vi "First.vi"(7 "Address":string, 8 "Error In":errorcluster) -> (0 "Error Out":errorcluster)   [LabVIEW 2018, in "Tests.lvlib" / "Known Hosts.lvlib"]
uses:
  Known Hosts.lvlib
  src/Toolkit/Known Hosts/Type Definitions/Get Results.ctl
  <vilib>/Utility/error.llb/Clear Errors.vi
  src/Toolkit/Known Hosts/Support/Create from Session.vi
  <vilib>/Utility/sysdir.llb/Get System Directory.vi
  src/Toolkit/Known Host/Support/Create from Known Hosts.vi
  src/Toolkit/Known Host/Support/Destroy to Known Hosts.vi
  src/Toolkit/Known Hosts/Support/Destroy to Session.vi
  <vilib>/addons/_JKI Toolkits/Caraya/classes/Test/Test.lvclass
  <vilib>/addons/_JKI Toolkits/Caraya/classes/Assert/Assert.lvclass
  src/Toolkit/Known Hosts/Known Hosts.lvclass
  Tests.lvlib
  src/Toolkit/Session/Session.lvclass
  src/Toolkit/Known Host/Known Host.lvclass
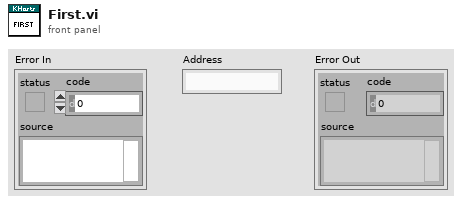
[diagram p1: front panel]
types:
  T1 = typedef "Toolkit.lvlib/Known Hosts.lvclass/Get Results.ctl" = i32
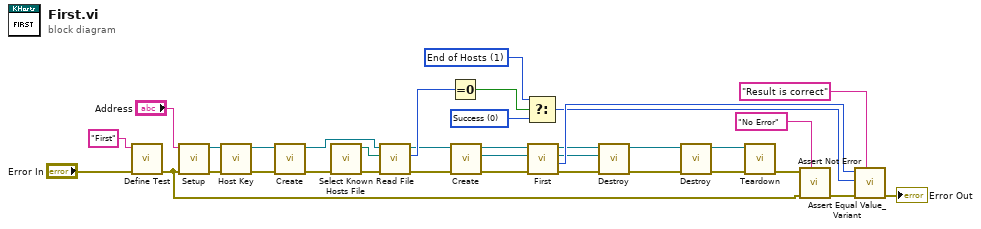
[diagram p0: block diagram]
diagram:
  w16 = T1 1 items=["Success", "End of Hosts"] ("Get Result")
  w17 = T1 0 items=["Success", "End of Hosts"] ("Get Result")
  n1 = call <vilib>:"Define Test.vi"("error in (no error)"="Error In", "Label (VI Title)"="First") -> ("error out"=w25:errorcluster)  [unwired: 9 in]
  n2 = call "Setup.vi"("Error In"=w25, "Address In"="Address") -> ("Error Out"=w26:errorcluster, "Sesssion"=w27:refnum<class "Session.lvclass">)  [unwired: 7 in, 1 out]
  n3 = call "Host Key.vi"("Error In"=w26, "Session In"=w27) -> ("Error Out"=w3:errorcluster, "Sesssion Out"=w4:refnum<class "Session.lvclass">)  [unwired: 6 in, 2 out]
  n4 = call-poly "Create.vi"("Error In"=w3, "Session"=w4) -> ("Error Out"=w2:errorcluster, "Known Hosts"=w1:refnum<class "Known Hosts.lvclass">)  [unwired: 8 in]
  n5 = call "Select Known Hosts File.vi"("Error In"=w2) -> ("Error Out"=w32:errorcluster, "Known Hosts File"=w31:path)  [unwired: 9 in]
  n6 = call "Read File.vi"("Error In"=w32, "File"=w31, "Known Hosts In"=w1) -> ("Error Out"=w22:errorcluster, "Count"=w19:u64, "Known Hosts Out"=w14:refnum<class "Known Hosts.lvclass">)  [unwired: 6 in]
  n7 = Equal To 0?(x=w19) -> (x = 0?=w18:bool)
  n8 = call-poly "Create.vi"("Error In"=w22, "Known Hosts In"=w14) -> ("Error Out"=w21:errorcluster, "Known Host"=w12:refnum<class "Known Host.lvclass">, "Known Hosts Out"=w13:refnum<class "Known Hosts.lvclass">)  [unwired: 7 in]
  n9 = Select(t=w16, s=w18, f=w17) -> (s? t:f=w15:T1)
  n10 = call "First.vi"("Error In"=w21, "Known Host In"=w12, "Known Hosts In"=w13) -> ("Error Out"=w9:errorcluster, "Result"=w20:T1, "Known Host Out"=w10:refnum<class "Known Host.lvclass">, "Known Hosts Out"=w11:refnum<class "Known Hosts.lvclass">)  [unwired: 5 in]
  n11 = call-poly "Destroy.vi"("Error In"=w9, "Known Host"=w10, "KnownHosts In"=w11) -> ("Error Out"=w5:errorcluster, "KnownHosts Out"=w8:refnum<class "Known Hosts.lvclass">)  [unwired: 7 in]
  n12 = call-poly "Destroy.vi"("Error In"=w5, "Known Hosts"=w8) -> ("Error Out"=w6:errorcluster, "Session"=w7:refnum<class "Session.lvclass">)  [unwired: 8 in]
  n13 = call "Teardown.vi"("Error In"=w6, "Session"=w7) -> ("Error Out"=w23:errorcluster)  [unwired: 9 in]
  n14 = call <vilib>:"Assert Not Error.vi"("Label"="No Error", "error in (no error)"=w25, "Not Error?"=w23) -> ("error out"=w30:errorcluster)  [unwired: 8 in]
  n15 = call <vilib>:"Assert Equal Value_Variant.vi"("Label"="Result is correct", "error in (no error)"=w30, "Y"=w15, "X"=w20) -> ("error out"=→"Error Out":errorcluster)  [unwired: 7 in]
